vi "update.description.request.vi"(8 "error in":errorcluster, 10 "description":string, 11 "event":refnum<class "event.lvclass">) -> (0 "error out":errorcluster, 3 "request":string)   [LabVIEW 2020, in "event.lvclass"]
uses:
  event.lvclass
  event.lvclass/event.ctl
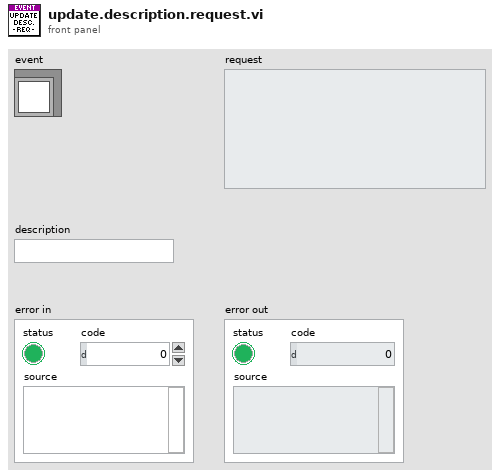
[diagram p1: front panel]
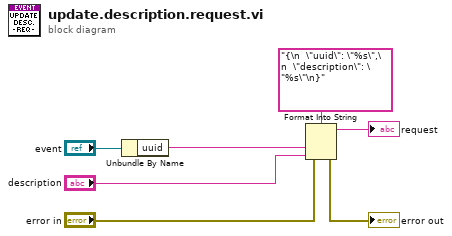
[diagram p0: block diagram]
diagram:
  n1 = Unbundle By Name("event") -> ("uuid"=w5:string)
  n2 = Format Into String(format string="{\n  \"uuid\": \"%s\",\n  \"description\": \"%s\"\n}", error in="error in", w5, "description") -> (resulting string=→"request":string, error out=→"error out":errorcluster)  [unwired: 1 in]
